vi "tp_filtre_010.vi"(8 "error in (no error)":errorcluster, 10 "ID Query (True)":bool=TRUE, 11 "VISA resource name":refnum<visa-resource-name>) -> ()   [LabVIEW 2012]
doc: "Establishes communication with the instrument and optionally performs an instrument identification query and/or an instrument reset. It also places the instrument in a default state needed for other instrument driver operations. Therefore, call this VI before calling other instrument driver VIs for this instrument. Generally, you need to call the <B>Initialize VI</B> only once at the beginning of an application."
panel:
  out "x = y? 2":bool
  out "concatenated string 2":string
  out "decimal integer string 2":string
  in  "Numeric 2":i32
  in  "VISA resource name 2":refnum<visa-resource-name>
  in  "ID Query (True) 2":bool=TRUE
  in  "error in (no error) 2":errorcluster
  out "decimal integer string":string
  out "concatenated string":string
  in  "Numeric":i32
  out "x = y?":bool
  # "(c) 2005-2008 National Instruments.  ALL RIGHTS RESERVED."
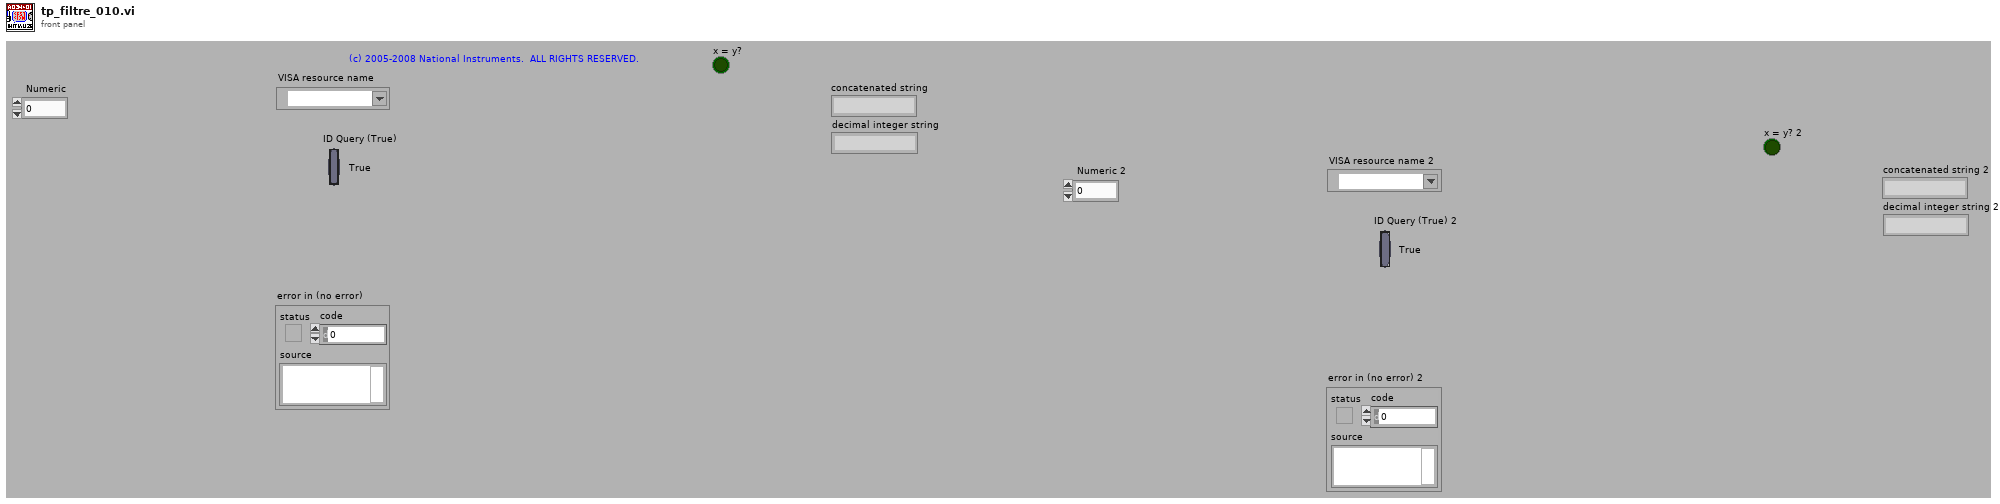
[diagram p1: front panel]
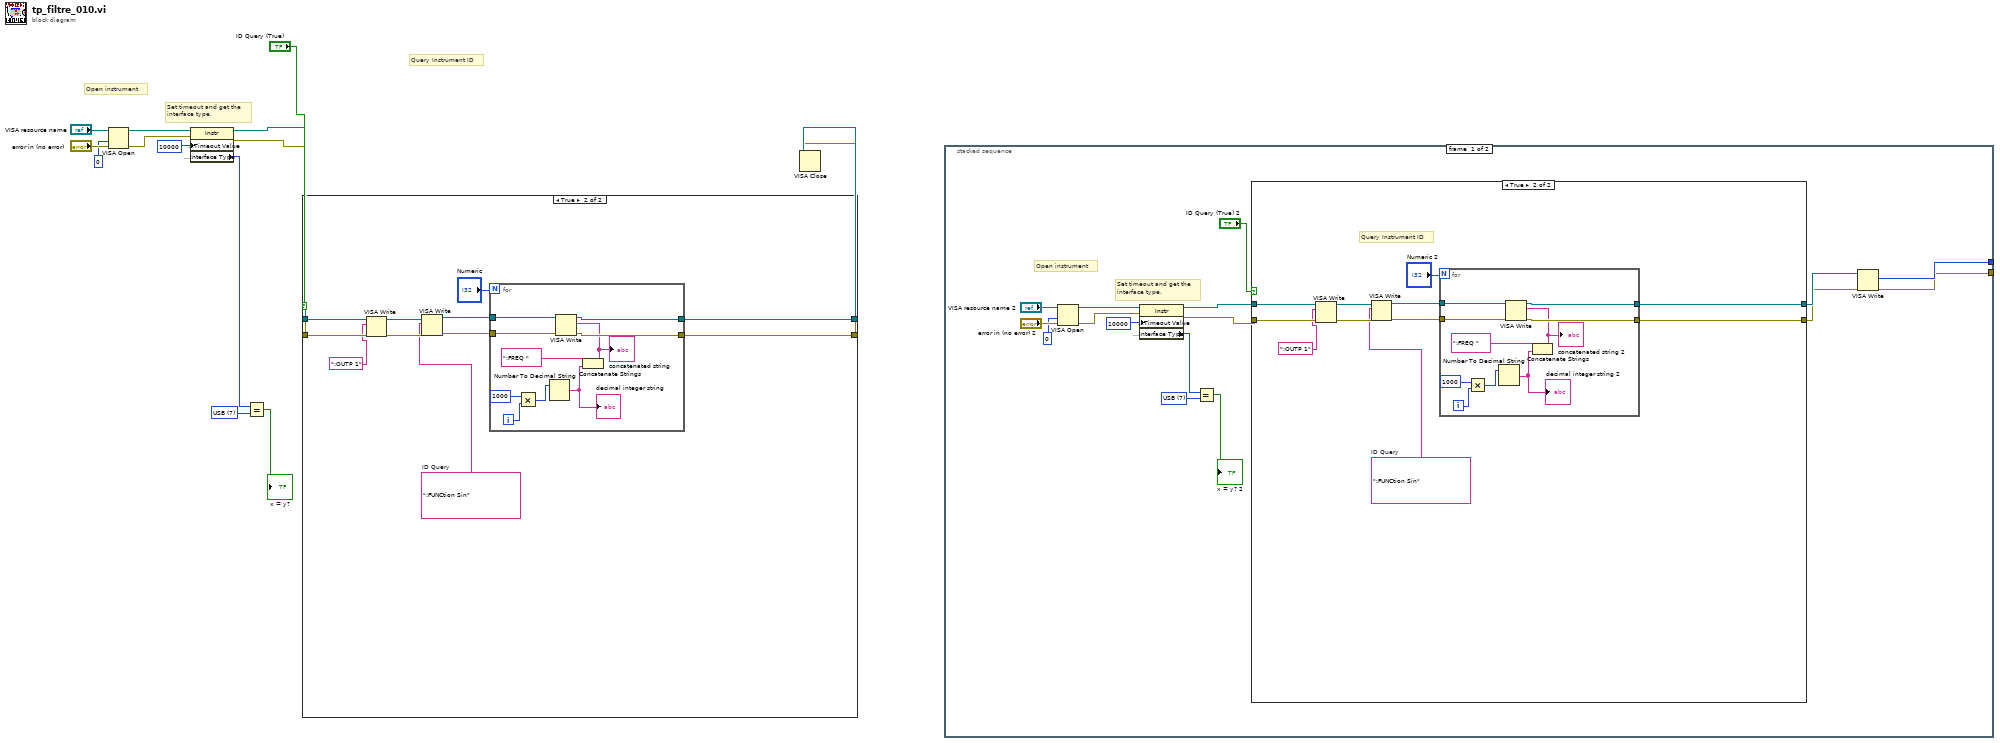
[diagram p0: block diagram]
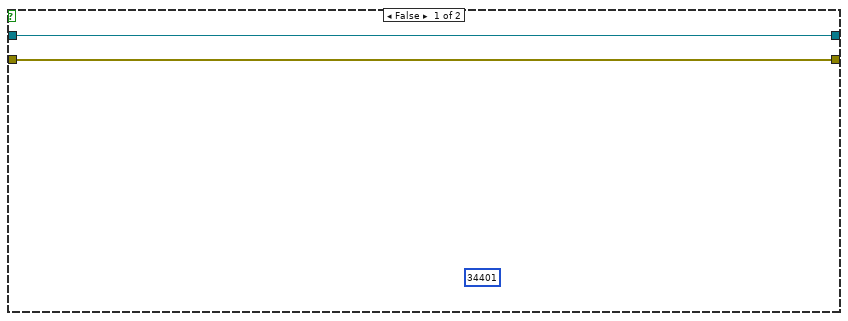
[diagram p2: hidden frame]
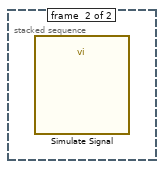
[diagram p3: hidden frame]
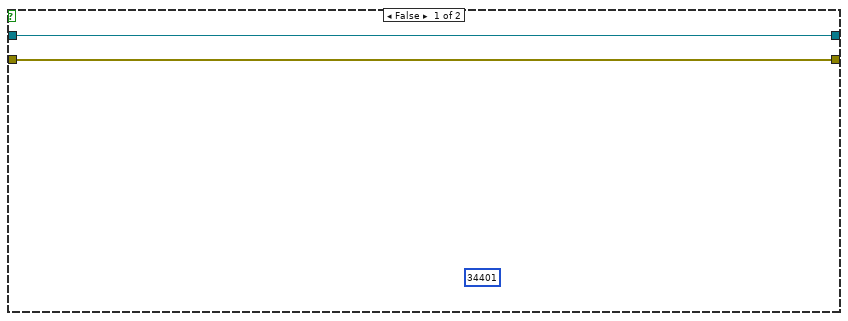
[diagram p4: hidden frame]
diagram:
  w10 = u16 7 items=["GPIB"=1, "VXI"=2, "GPIB-VXI"=3, "Serial"=4, "PXI"=5, "TCPIP"=6, "USB"=7] ("Interface Information:Interface Type")
  # "Set timeout and get the\ninterface type."
  # "Query Instrument ID"
  # "Open instrument"
  n1 = VISA Open(access mode=u32 0, error in (no error)="error in (no error)", VISA resource name="VISA resource name") -> (VISA resource name=w7:refnum<visa-resource-name>, error out=w6:errorcluster)  [unwired: 2 in]
  n2 = property on="Property Node" class="Instr"(reference=w7, error in=w6, "General Settings:Timeout Value"=u32 10000) -> (reference out=w5:refnum<visa-resource-name>, error out=w4:errorcluster, "Interface Information:Interface Type"=w12:u16)
  n3 = Equal?(x=w12, y=w10) -> (x = y?=→"x = y?":bool)
  n4 = case shown="True" "ID Query (True)" {
    tunnel: [w15 w19] -> w1
    tunnel: [w16 w20] -> w2
    tunnel: w5 -> [w16 w26]
    tunnel: w4 -> [w15 w27]
    frame False {
      (unwired) 34401
    }
    frame True {
      w23 = ":FUNCtion Sin"  # ID Query
      n5 = VISA Write(VISA resource name=w26, write buffer=":OUTP 1", error in (no error)=w27) -> (VISA resource name out=w25:refnum<visa-resource-name>, error out=w24:errorcluster)  [unwired: 1 out]
      n6 = VISA Write(VISA resource name=w25, write buffer=w23, error in (no error)=w24) -> (VISA resource name out=w22:refnum<visa-resource-name>, error out=w21:errorcluster)  [unwired: 1 out]
      n7 = for {
        N: "Numeric" -> [_]
        tunnel: w22 -> [w37]
        tunnel: w21 -> [w36]
        tunnel: [w34] -> w20
        tunnel: [w33] -> w19
        i -> [w29]
        n8 = Multiply(x=1000, y=w29) -> (x*y=w30:i32)
        n9 = Number To Decimal String(number=w30) -> (decimal integer string=w31:string)  [unwired: 1 in]
        "decimal integer string" <- w31
        n10 = Concatenate Strings(":FREQ ", w31) -> (w32:string)
        "concatenated string" <- w32
        n11 = VISA Write(VISA resource name=w37, write buffer=w32, error in (no error)=w36) -> (VISA resource name out=w34:refnum<visa-resource-name>, error out=w33:errorcluster)  [unwired: 1 out]
      }
    }
  }
  n12 = VISA Close(VISA resource name=w2, error in (no error)=w1) -> ()  [unwired: 1 out]
  n13 = stacked-sequence {
    tunnel: [w39 _] -> _
    tunnel: [w38 _] -> _
    frame #0 {
      w49 = u16 7 items=["GPIB"=1, "VXI"=2, "GPIB-VXI"=3, "Serial"=4, "PXI"=5, "TCPIP"=6, "USB"=7] ("Interface Information:Interface Type")
      # "Set timeout and get the\ninterface type."
      # "Query Instrument ID"
      # "Open instrument"
      n14 = VISA Open(access mode=u32 0, error in (no error)="error in (no error) 2", VISA resource name="VISA resource name 2") -> (VISA resource name=w46:refnum<visa-resource-name>, error out=w45:errorcluster)  [unwired: 2 in]
      n15 = property on="Property Node" class="Instr"(reference=w46, error in=w45, "General Settings:Timeout Value"=u32 10000) -> (reference out=w44:refnum<visa-resource-name>, error out=w43:errorcluster, "Interface Information:Interface Type"=w51:u16)
      n16 = Equal?(x=w51, y=w49) -> (x = y?=→"x = y? 2":bool)
      n17 = case shown="True" "ID Query (True) 2" {
        tunnel: [w54 w58] -> w40
        tunnel: [w55 w59] -> w41
        tunnel: w44 -> [w55 w65]
        tunnel: w43 -> [w54 w66]
        frame False {
          (unwired) 34401
        }
        frame True {
          w62 = ":FUNCtion Sin"  # ID Query
          n18 = VISA Write(VISA resource name=w65, write buffer=":OUTP 1", error in (no error)=w66) -> (VISA resource name out=w64:refnum<visa-resource-name>, error out=w63:errorcluster)  [unwired: 1 out]
          n19 = VISA Write(VISA resource name=w64, write buffer=w62, error in (no error)=w63) -> (VISA resource name out=w61:refnum<visa-resource-name>, error out=w60:errorcluster)  [unwired: 1 out]
          n20 = for {
            N: "Numeric 2" -> [_]
            tunnel: w61 -> [w76]
            tunnel: w60 -> [w75]
            tunnel: [w73] -> w59
            tunnel: [w72] -> w58
            i -> [w68]
            n21 = Multiply(x=1000, y=w68) -> (x*y=w69:i32)
            n22 = Number To Decimal String(number=w69) -> (decimal integer string=w70:string)  [unwired: 1 in]
            "decimal integer string 2" <- w70
            n23 = Concatenate Strings(":FREQ ", w70) -> (w71:string)
            "concatenated string 2" <- w71
            n24 = VISA Write(VISA resource name=w76, write buffer=w71, error in (no error)=w75) -> (VISA resource name out=w73:refnum<visa-resource-name>, error out=w72:errorcluster)  [unwired: 1 out]
          }
        }
      }
      n25 = VISA Write(VISA resource name=w41, error in (no error)=w40) -> (return count=w39:u32, error out=w38:errorcluster)  [unwired: 1 in, 1 out]
    }
    frame #1 {
      n26 = call "Simulate Signal"() -> ()  [unwired: 14 in, 2 out]
    }
  }
